vi "write_table_key_string.vi"(7 "table":string="nipm", 8 "error in (no error)":errorcluster, 9 "value":string="6.6.6", 10 "key":string="version", 11 "toml in":refnum<class "toml.lvclass">) -> (0 "error out":errorcluster, 3 "toml out":refnum<class "toml.lvclass">)   [LabVIEW 2020, in "toml.lvclass"]
uses:
  toml.lvclass
  toml.lvclass/toml.ctl
  Item/Item.lvclass
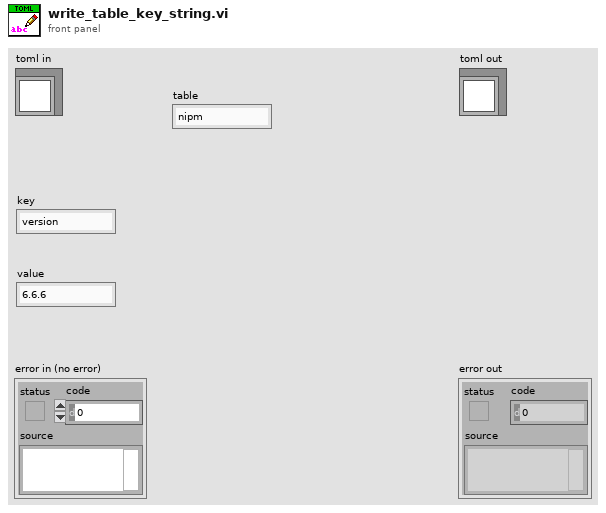
[diagram p1: front panel]
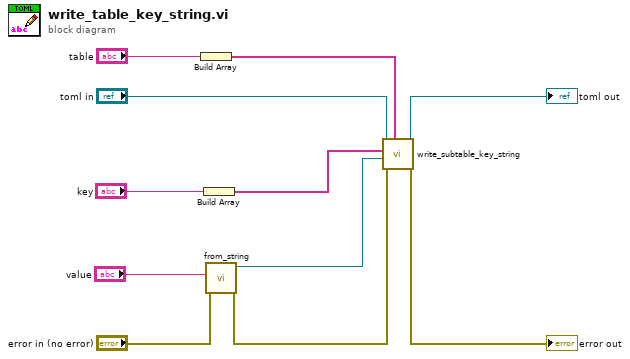
[diagram p0: block diagram]
diagram:
  n1 = Build Array("table") -> (w6:string[])
  n2 = Build Array("key") -> (w5:string[])
  n3 = call "from_string.vi"("error in (no error)"="error in (no error)", "string"="value") -> ("error out"=w1:errorcluster, "Item out"=w3:refnum<class "Item.lvclass">)  [unwired: 8 in]
  n4 = call "write_subtable_key_string.vi"("subtables"=w6, "error in (no error)"=w1, "Item"=w3, "subkeys"=w5, "toml in"="toml in") -> ("error out"=→"error out":errorcluster, "toml out"=→"toml out":refnum<class "toml.lvclass">)  [unwired: 5 in]
